vi "Get SubVI Dependencies.vi"(0 "dependency paths":path[](array[path]), 11 "error in":errorcluster) -> (4 "all dependencies":path[](array[path]), 6 "instrument containing sub vis":path[](array[path]), 15 "error out":errorcluster)   [LabVIEW 2021, in "Multiple Converter.lvlib"]
uses:
  Multiple Converter.lvlib
  Converter Reusables/Converter Reusables.lvlib
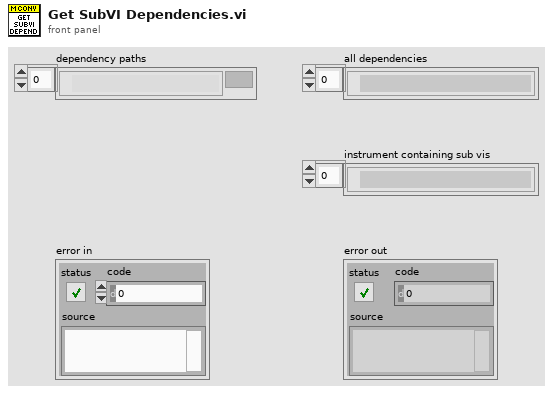
[diagram p1: front panel]
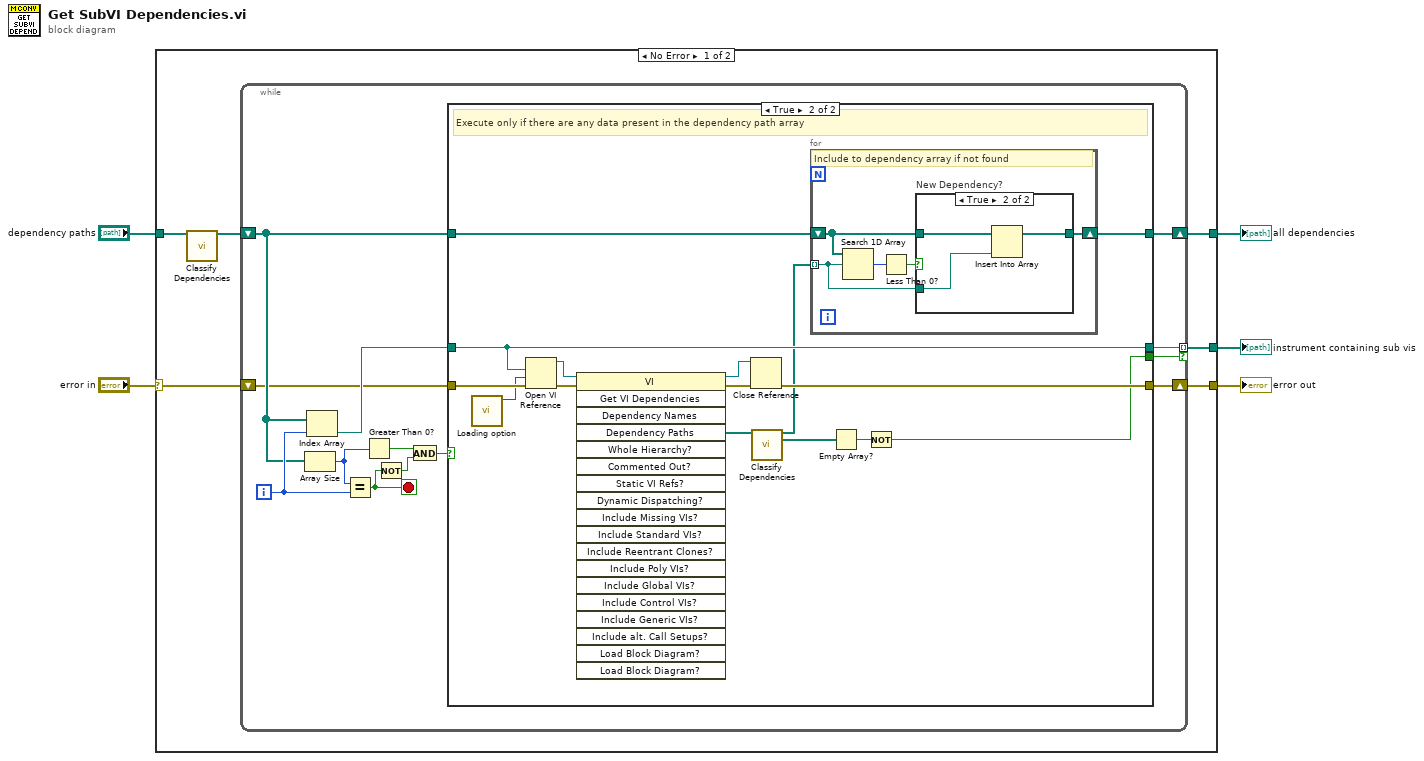
[diagram p0: block diagram]
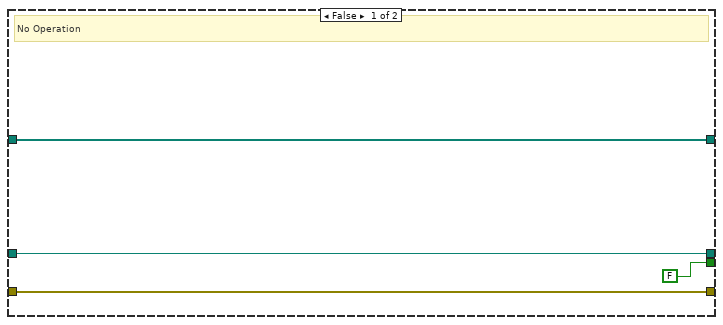
[diagram p2: hidden frame]
diagram:
  n1 = case shown="No Error" "error in" {
    selector: "error in" -> [w10 w53]
    tunnel: [w11 w53] -> w5
    tunnel: [w9 _] -> w3
    tunnel: "dependency paths" -> [w7 _]
    tunnel: [w6 _] -> w1
    frame No Error {
      n2 = call "Classify Dependencies.vi"("dependency paths"=w7) -> ("actual dependencies"=w8:path[])  [unwired: 13 in, 1 out]
      n3 = while {
        shift-right: [w22] -> w9
        shift-left: w8 -> [w23]
        shift-right: [w19] -> w11
        shift-left: w10 -> [w20]
        tunnel: [w13] -> w6 mode=indexing if=w12
        i -> [w24]
        stop <- w17 stop-if-true
        n4 = Array Size(array=w23) -> (size(s)=w18:i32)
        n5 = Index Array(array=w23, index=w24) -> (element=w21:path)
        n6 = Equal?(x=w18, y=w24) -> (x = y?=w17:bool)
        n7 = Greater Than 0?(x=w18) -> (x > 0?=w15:bool)
        n8 = Not(x=w17) -> (.not. x?=w14:bool)
        n9 = And(x=w15, y=w14) -> (x .and. y?=w16:bool)
        n10 = case shown="True" w16 {
          tunnel: w23 -> [w27 w41]
          tunnel: [w27 w40] -> w22
          tunnel: w21 -> [w26 w35]
          tunnel: w20 -> [w28 w39]
          tunnel: [w28 w38] -> w19
          tunnel: [w26 w35] -> w13
          tunnel: [FALSE w34] -> w12
          frame False {
            # "No Operation"
          }
          frame True {
            # "Execute only if there are any data present in the dependency path array"
            n11 = call "Loading option.vi"() -> ("options"=w29:i32)  [unwired: 11 in]
            n12 = Open VI Reference(vi path=w35, options=w29, error in (no error)=w39) -> (vi reference=w42:refnum<vi>, error out=w43:errorcluster)  [unwired: 3 in]
            n13 = invoke class="VI" method="Get VI Dependencies"(reference=w42, error in=w43) -> (reference out=w33:refnum<vi>, error out=w32:errorcluster, "Dependency Paths"=w31:path[])  [unwired: 17 in, 16 out]
            n14 = Close Reference(reference=w33, error in (no error)=w32) -> (error out=w38:errorcluster)
            n15 = call "Classify Dependencies.vi"("dependency paths"=w31) -> ("actual dependencies"=w30:path[], "driver vis"=w37:path[])  [unwired: 13 in]
            n16 = for {
              tunnel: w30 -> [w45] mode=indexing
              shift-right: [w44] -> w40
              shift-left: w41 -> [w46]
              # "Include to dependency array if not found"
              n17 = Search 1D Array(1D array=w46, element=w45) -> (index of element=w48:i32)  [unwired: 1 in]
              n18 = Less Than 0?(x=w48) -> (x < 0?=w47:bool)
              n19 = case "New Dependency?" shown="True" w47 {
                tunnel: w46 -> [w49 w52]
                tunnel: w45 -> [_ w51]
                tunnel: [w49 w50] -> w44
                frame False {
                }
                frame True {
                  n20 = Insert Into Array(array=w52, new element=w51) -> (w50:path[])  [unwired: 1 in]
                }
              }
            }
            n21 = Empty Array?(array=w37) -> (empty?=w36:bool)
            n22 = Not(x=w36) -> (.not. x?=w34:bool)
          }
        }
      }
    }
    frame Error {
    }
  }
  "error out" <- w5
  "all dependencies" <- w3
  "instrument containing sub vis" <- w1
